vi "Open_All.vi"(8 "error in (no error)":errorcluster) -> (0 "error out":errorcluster, 1 "Modbus out":refnum<k5>, 2 "Motion out":refnum<visa-resource-name>, 3 "Camera out":refnum<k5>)   [LabVIEW 2018]
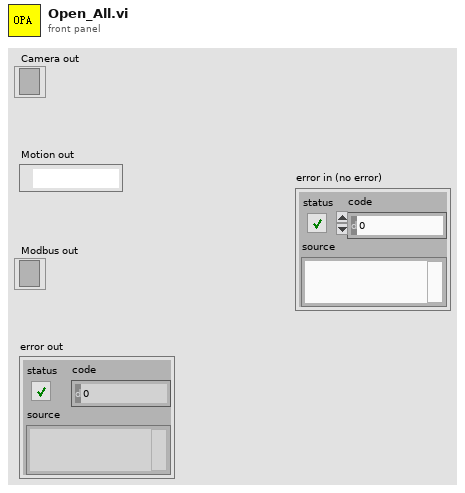
[diagram p1: front panel]
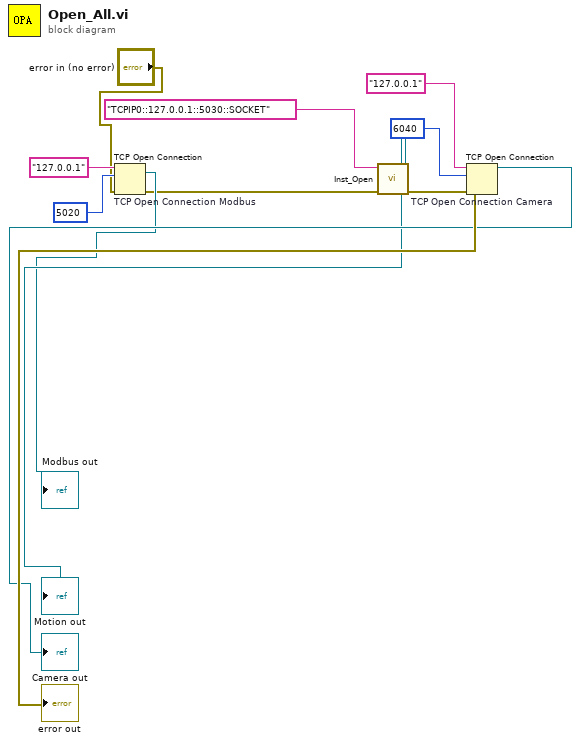
[diagram p0: block diagram]
diagram:
  n1 = TCP Open Connection "TCP Open Connection Modbus"(address="127.0.0.1", remote port or service name=u16 5020, error in (no error)="error in (no error)") -> (connection ID=→"Modbus out":refnum<k5>, error out=w7:errorcluster)  [unwired: 2 in]
  n2 = call "Inst_Open.vi"("error in (no error)"=w7, "VISA Refnum in"="TCPIP0::127.0.0.1::5030::SOCKET" ("address")) -> ("error out"=w8:errorcluster, "VISA Refnum out"=→"Motion out":refnum<visa-resource-name>)  [unwired: 8 in]
  n3 = TCP Open Connection "TCP Open Connection Camera"(address="127.0.0.1", remote port or service name=u16 6040, error in (no error)=w8) -> (connection ID=→"Camera out":refnum<k5>, error out=→"error out":errorcluster)  [unwired: 2 in]
